vi "List States in Category.vi"(8 "error in (no error)":errorcluster, 10 "Category":string, 11 "JKI SM in":refnum<class "JKI SM.lvclass">) -> (0 "error out":errorcluster, 1 "State Frame Indices":i32[](array[numeric]), 2 "States":string[](array[string]), 3 "JKI SM out":refnum<class "JKI SM.lvclass">, 4 "Category Frame Index":i32)   [LabVIEW 2020, in "JKI State Machine API.lvlib" / "JKI SM.lvclass"]
uses:
  JKI SM.lvclass
  JKI SM.lvclass/JKI SM.ctl
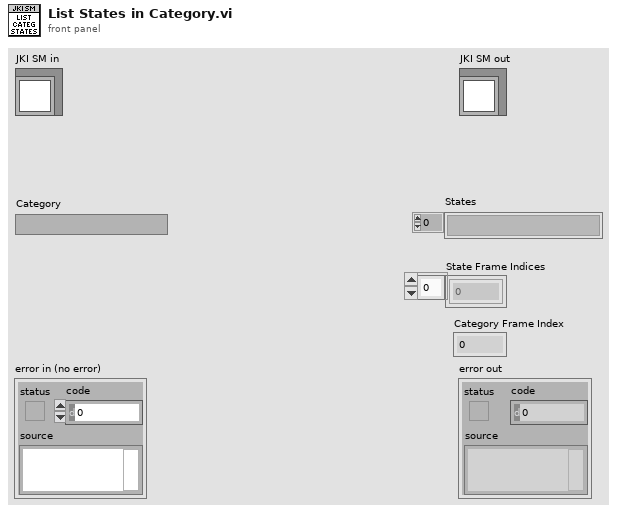
[diagram p1: front panel]
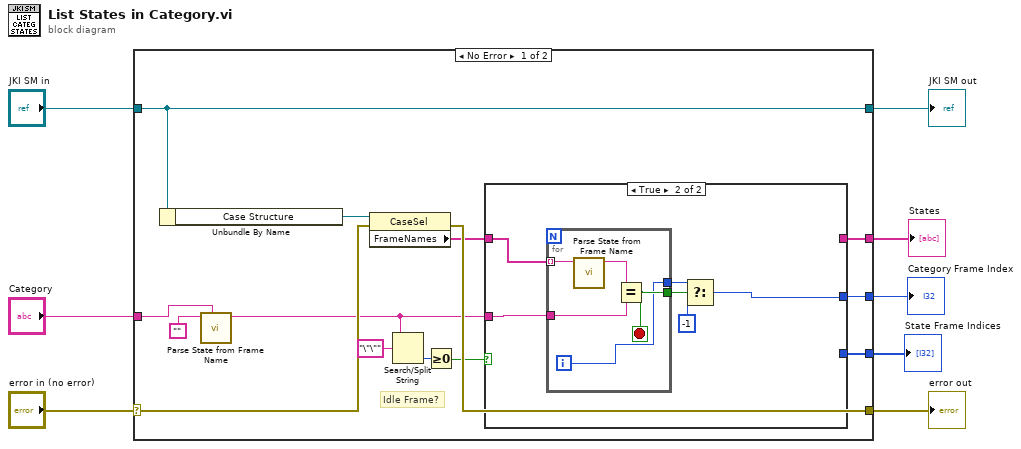
[diagram p0: block diagram]
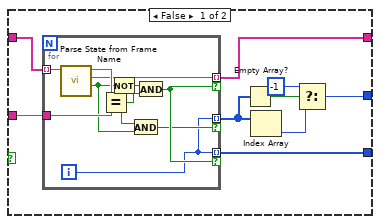
[diagram p2: hidden frame]
diagram:
  n1 = case shown="No Error" "error in (no error)" {
    selector: "error in (no error)" -> [w20 w54]
    tunnel: [w19 w54] -> w7
    tunnel: [w22 w53] -> w5
    tunnel: "JKI SM in" -> [w22 w53]
    tunnel: [w17 _] -> w4
    tunnel: "Category" -> [w14 _]
    tunnel: [w16 _] -> w2
    tunnel: [w15 _] -> w1
    frame No Error {
      # "Idle Frame?"
      n2 = Unbundle By Name(w22) -> ("Case Structure"=w21:refnum<vi>)
      n3 = call "Parse State from Frame Name.vi"("Category (Optional)"=w14, "Frame or State Name"="") -> ("Category Name"=w12:string)  [unwired: 4 in, 5 out]
      n4 = property class="CaseSel"(reference=w21, error in=w20) -> (error out=w19:errorcluster, "FrameNames"=w18:string[])  [unwired: 1 out]
      n5 = Search/Split String(string=w12, search string/char (-)="\"\"") -> (offset of match=w10:i32)  [unwired: 1 in, 2 out]
      n6 = Greater Or Equal To 0?(x=w10) -> (x >= 0?=w9:bool)
      n7 = case shown="True" w9 {
        tunnel: w18 -> [w31 w47]
        tunnel: [w30 _] -> w17
        tunnel: [w29 _] -> w16
        tunnel: [w24 w42] -> w15
        tunnel: w12 -> [w23 w46]
        frame False {
          n8 = for {
            tunnel: w23 -> [w39]
            tunnel: w31 -> [w41] mode=indexing
            tunnel: [w38] -> w30 mode=indexing if=w36
            tunnel: [w32] -> w29 mode=indexing if=w36
            tunnel: [w32] -> w28 mode=indexing if=w33
            i -> [w32]
            n9 = call "Parse State from Frame Name.vi"("Frame or State Name"=w41) -> ("is a Category Frame?"=w34:bool, "State Name"=w38:string, "Category Name"=w40:string)  [unwired: 5 in, 3 out]
            n10 = Equal?(x=w40, y=w39) -> (x = y?=w35:bool)
            n11 = Not(x=w34) -> (.not. x?=w37:bool)
            n12 = And(x=w35, y=w34) -> (x .and. y?=w33:bool)
            n13 = And(x=w37, y=w35) -> (x .and. y?=w36:bool)
          }
          n14 = Empty Array?(array=w28) -> (empty?=w27:bool)
          n15 = Index Array(array=w28) -> (element=w26:i32)  [unwired: 1 in]
          n16 = Select(t=-1, s=w27, f=w26) -> (s? t:f=w24:i32)
        }
        frame True {
          n17 = for {
            tunnel: w47 -> [w52] mode=indexing
            tunnel: w46 -> [w50]
            tunnel: [w49] -> w45
            tunnel: [w48] -> w44
            i -> [w48]
            stop <- w49 stop-if-true
            n18 = call "Parse State from Frame Name.vi"("Frame or State Name"=w52) -> ("Category Name"=w51:string)  [unwired: 5 in, 5 out]
            n19 = Equal?(x=w51, y=w50) -> (x = y?=w49:bool)
          }
          n20 = Select(t=w44, s=w45, f=-1) -> (s? t:f=w42:i32)
        }
      }
    }
    frame Error {
    }
  }
  "error out" <- w7
  "JKI SM out" <- w5
  "States" <- w4
  "State Frame Indices" <- w2
  "Category Frame Index" <- w1
